vi "Measurement data to delimited string - SubVI.vi"(6 "Measurement data":dbl[][](array[numeric]), 9 "Header title string":string[][](array[string]), 10 "Header format string":string, 11 "Delimiter in":string) -> (3 "File string out":string)   [LabVIEW 2025]
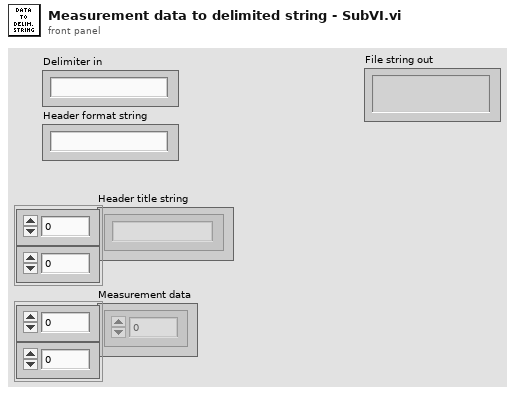
[diagram p1: front panel]
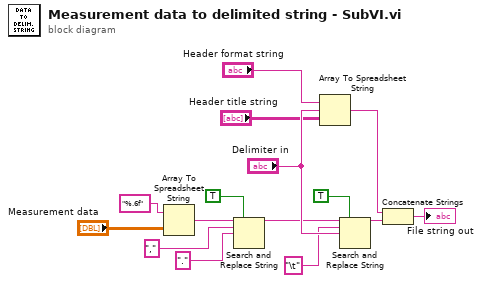
[diagram p0: block diagram]
diagram:
  n1 = Array To Spreadsheet String(array="Measurement data", 3:"%.6f" ("format string")) -> (spreadsheet string=w9:string)  [unwired: 1 in]
  n2 = Search and Replace String(replace all?=TRUE ("replace all? (F)"), input string=w9, search string=",", replace string="." ("replace string (\"\")")) -> (result string=w12:string)  [unwired: 4 in, 3 out]
  n3 = Array To Spreadsheet String(delimiter (Tab)="Delimiter in", array="Header title string", 3:"Header format string") -> (spreadsheet string=w4:string)
  n4 = Search and Replace String(replace all?=TRUE ("replace all? (F)"), input string=w12, search string="\t", replace string="Delimiter in") -> (result string=w15:string)  [unwired: 4 in, 3 out]
  n5 = Concatenate Strings(w4, w15) -> (→"File string out":string)
